vi "Update_Result.vi"(8 "error in (no error) 2":errorcluster, 11 "Boolean":bool=TRUE) -> (0 "error in (no error) 3":errorcluster, 1 "FAIL":string, 2 "PASS":string, 3 "TOTAL":string)   [LabVIEW 2021]
uses:
  Template/Main_VI/Control/Ini.ctl
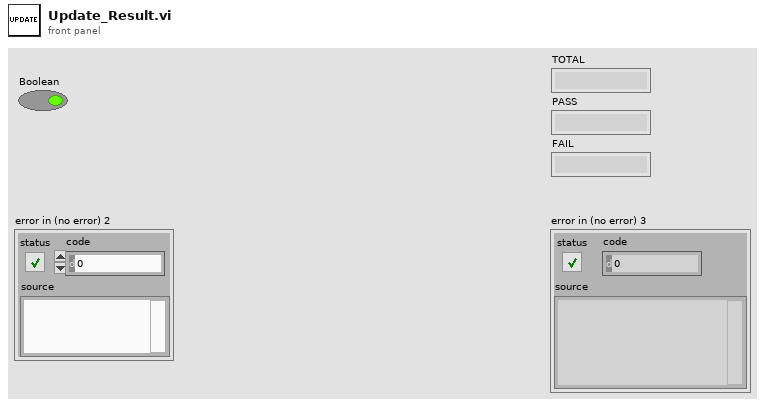
[diagram p1: front panel]
types:
  T1 = typedef "Ini.ctl" = enum16{"Write", "Read"}
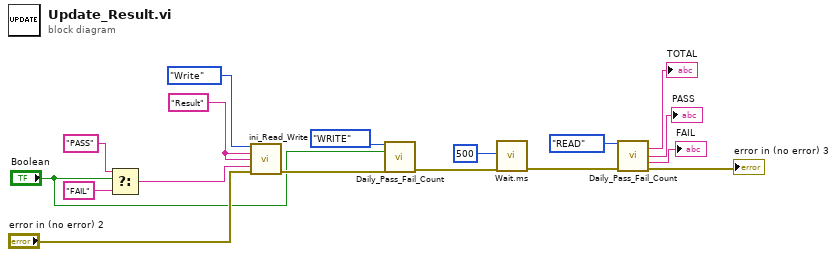
[diagram p0: block diagram]
diagram:
  w16 = "Result" ("Read Section")
  n1 = Select(t="PASS" ("Write"), s="Boolean", f="FAIL") -> (s? t:f=w12:string)
  n2 = call "ini_Read_Write.vi"(0:Ini."Write", "Write Section"=w16, "Write key"=w16, "Write"=w12, "error in (no error) 2"="error in (no error) 2") -> ("error in (no error) 3"=w11:errorcluster)  [unwired: 9 in, 1 out]
  n3 = call "Daily_Pass_Fail_Count.vi"("Action"=enum16{"READ", "WRITE"}."WRITE", "Result"="Boolean", "error in"=w11) -> ("error out"=w5:errorcluster)  [unwired: 7 in, 5 out]
  n4 = call "Wait.ms.vi"("error in"=w5, "milliseconds to wait"=u32 500) -> ("error out"=w4:errorcluster)  [unwired: 9 in]
  n5 = call "Daily_Pass_Fail_Count.vi"("Action"=enum16{"READ", "WRITE"}."READ", "error in"=w4) -> ("TOTAL"=→"TOTAL":string, "PASS"=→"PASS":string, "FAIL"=→"FAIL":string, "error out"=→"error in (no error) 3":errorcluster)  [unwired: 8 in, 2 out]
